vi "fix_shared_library_paths_for_folder.vi"(8 "error in":errorcluster, 11 "Folder of VIs":path=path "C:/Projects/reqwest-rs-labview/jki_lib_reqwest_rs_labview-0.1.0.1/File Group 0/vi.lib/JKI/reqwest-rs-labview") -> (0 "error out":errorcluster, 2 "map of replacements":map{path, path}(c390))   [LabVIEW 2020, in "vi_package_building_extensions.lvlib" / "fix_shared_library_wildcards.lvlib"]
uses:
  fix_shared_library_wildcards.lvlib
  <vilib>/Utility/traverseref.llb/TRef TravTarget.ctl
  <vilib>/Utility/traverseref.llb/VI Scripting - Traverse.lvlib
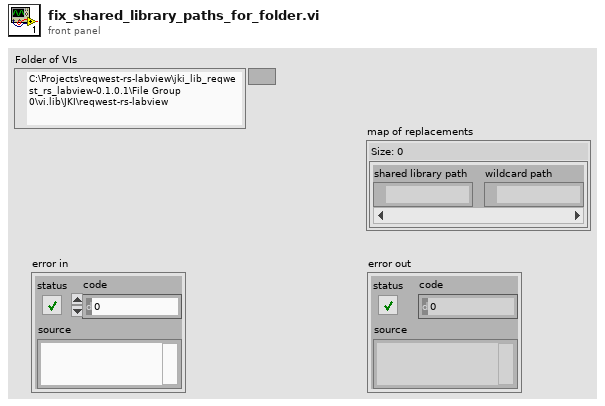
[diagram p1: front panel]
types:
  T1 = typedef "TRef TravTarget.ctl" = enum16{"FP", "BD", "Other"}
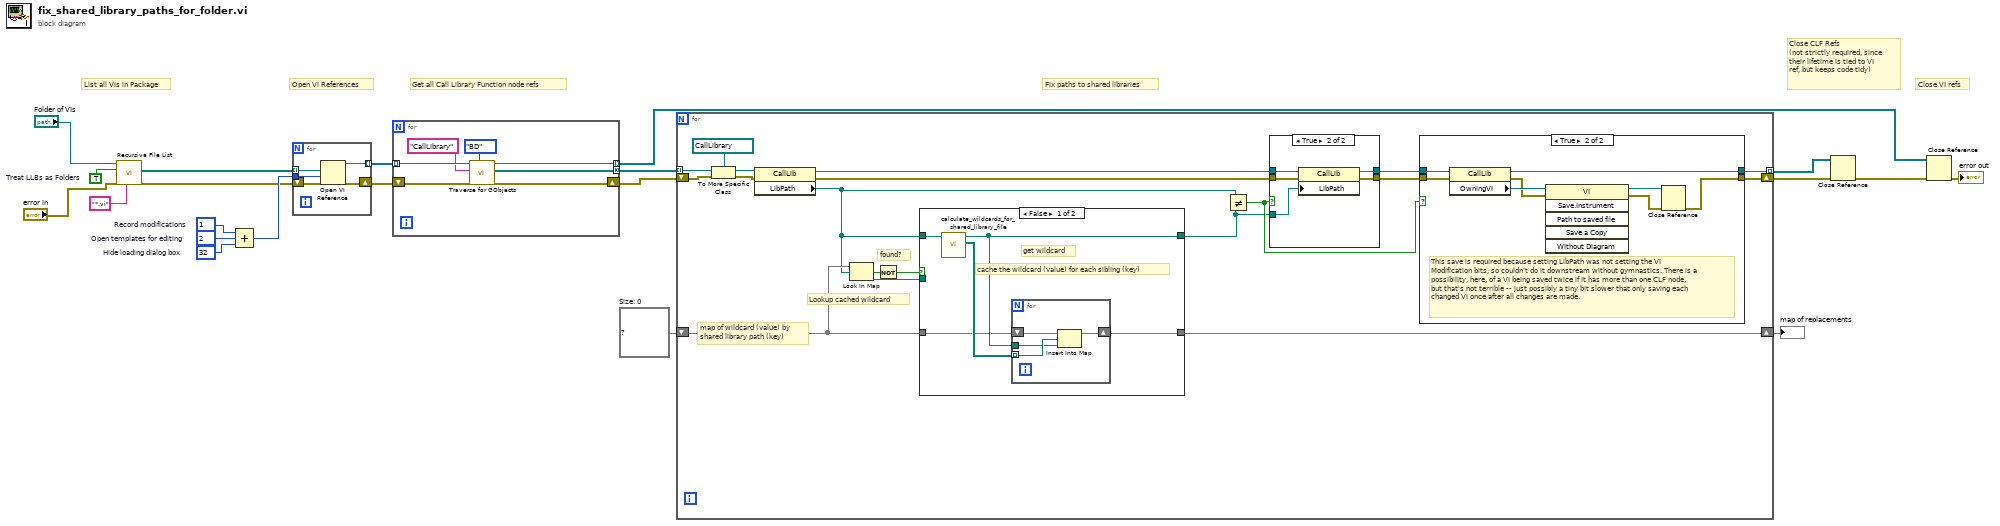
[diagram p0: block diagram]
diagram:
  w2 = map{path, path} {}  # Size: 0
  w13 = 32  # Hide loading dialog box
  w15 = 2  # Open templates for editing
  w14 = 1  # Record modifications
  w21 = TRUE  # Treat LLBs as Folders
  # "Close CLF Refs\n(not strictly required, since their lifetime is tied to VI ref, but keeps code tidy)"
  # "Close VI refs"
  # "List all VIs in Package"
  # "Open VI References"
  # "Fix paths to shared libraries"
  # "Get all Call Library Function node refs"
  n1 = call <vilib>:"Recursive File List.vi"("pattern"="*.vi", "error in (no error)"="error in", "Treat LLBs as Folders?"=w21, "Folder Path"="Folder of VIs") -> ("error out"=w9:errorcluster, "All Files in Dir"=w19:path[])  [unwired: 3 in, 3 out]
  n2 = Compound Arithmetic op=unknown(w14, w15, w13) -> (w12:i32)
  n3 = for {
    tunnel: w19 -> [w26] mode=indexing
    tunnel: [w25] -> w18 mode=indexing
    tunnel: w12 -> [w24]
    shift-right: [w23] -> w10
    shift-left: w9 -> [w22]
    n4 = Open VI Reference(vi path=w26, options=w24, error in (no error)=w22) -> (vi reference=w25:refnum<vi>, error out=w23:errorcluster)  [unwired: 3 in]
  }
  n5 = for {
    tunnel: w18 -> [w33] mode=indexing
    tunnel: [w31] -> w17 mode=concatenating
    tunnel: [w29] -> w16 mode=indexing
    shift-right: [w28] -> w11
    shift-left: w10 -> [w27]
    n6 = call <vilib>:"Traverse for GObjects.vi"("Traverse Target"=TRef_TravTarget."BD", "error in (no error)"=w27, "Class Name"="CallLibrary", "VI Refnum"=w33) -> ("error out"=w28:errorcluster, "References"=w31:refnum<vi>[], "dup VI Refnum"=w29:refnum<vi>)  [unwired: 4 in, 1 out]
  }
  n7 = for {
    tunnel: w17 -> [w52] mode=indexing
    shift-right: [w44] -> w7
    shift-left: w11 -> [w47]
    tunnel: [w42] -> w8 mode=indexing
    shift-right: [w40] -> w1
    shift-left: w2 -> [w39]
    # "Lookup cached wildcard"
    # "map of wildcard (value) by shared library path (key)"
    # "found?"
    n8 = To More Specific Class(target class=refnum<vi> refnum ("Other Refnum"), reference=w52, error in=w47) -> (specific class reference=w50:refnum<vi>, error out=w46:errorcluster)
    n9 = property class="CallLib"(reference=w50, error in=w46) -> (reference out=w49:refnum<vi>, error out=w48:errorcluster, "LibPath"=w38:path)
    n10 = Look In Map(map=w39, key=w38) -> (key not found?=w37:bool, value=w36:path)  [unwired: 1 in]
    n11 = Not(x=w37) -> (.not. x?=w35:bool)
    n12 = case shown="False" w35 {
      tunnel: [w56 w63] -> w34
      tunnel: [w55 w62] -> w40
      tunnel: w39 -> [w54 w62]
      tunnel: w38 -> [w53 _]
      tunnel: w36 -> [_ w63]
      frame False {
        # "cache the wildcard (value) for each sibling (key)"
        # "get wildcard"
        n13 = call "calculate_wildcards_for_shared_library_file.vi"("Shared Library Path"=w53) -> ("sibling shared libraries"=w57:path[], "Shared Library Path with wildcards"=w56:path)  [unwired: 8 in, 1 out]
        n14 = for {
          tunnel: w57 -> [w61] mode=indexing
          tunnel: w56 -> [w60]
          shift-right: [w59] -> w55
          shift-left: w54 -> [w58]
          n15 = Insert Into Map(map in=w58, key=w61, value=w60) -> (map out=w59:map{path, path})  [unwired: 2 out]
        }
      }
      frame True {
        # "use cached value"
      }
    }
    n16 = Not Equal?(x=w38, y=w34) -> (x != y?=w41:bool)
    n17 = case shown="True" w41 {
      tunnel: w49 -> [w75 w80]
      tunnel: [w74 w77] -> w45
      tunnel: w48 -> [w74 w79]
      tunnel: [w75 w76] -> w43
      tunnel: w34 -> [_ w78]
      frame False {
      }
      frame True {
        n18 = property class="CallLib"(reference=w80, error in=w79, "LibPath"=w78) -> (reference out=w76:refnum<vi>, error out=w77:errorcluster)
      }
    }
    n19 = case shown="True" w41 {
      tunnel: w43 -> [w65 w73]
      tunnel: [w64 w67] -> w44
      tunnel: w45 -> [w64 w72]
      tunnel: [w65 w66] -> w42
      frame False {
      }
      frame True {
        # "This save is required because setting LibPath was not setting the VI Modification bits, so couldn't do it downstream without gymnastics. There is a possibility, here, of a VI being saved twice if it has more than one CLF node, but that's not terrible -- just possibly a tiny bit slower that only saving each changed VI once after all changes are made."
        n20 = property class="CallLib"(reference=w73, error in=w72) -> (reference out=w66:refnum<vi>, error out=w68:errorcluster, "OwningVI"=w71:refnum<vi>)
        n21 = invoke class="VI" method="Save.Instrument"(reference=w71, error in=w68) -> (reference out=w69:refnum<vi>, error out=w70:errorcluster)  [unwired: 4 in, 4 out]
        n22 = Close Reference(reference=w69, error in (no error)=w70) -> (error out=w67:errorcluster)
      }
    }
  }
  "map of replacements" <- w1
  n23 = Close Reference(reference=w8, error in (no error)=w7) -> (error out=w6:errorcluster)
  n24 = Close Reference(reference=w16, error in (no error)=w6) -> (error out=→"error out":errorcluster)
